vi "helper_fp_print.vi"(1 "VI Path":string, 2 "HTML File Path":string, 3 "Image Directory":string) -> (0 "status":bool, 4 "code":i32, 5 "source":string)   [LabVIEW 2026]
doc: "Print one VI's FRONT PANEL to an HTML file with PNG images. Driven by RunVIAsTopLevel, which can only set STRING controls - paths are built on the diagram."
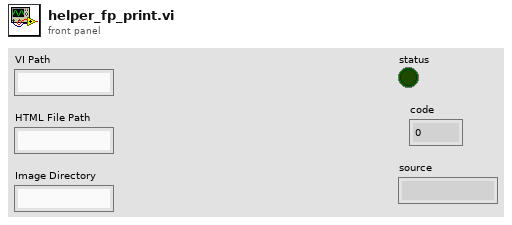
[diagram p1: front panel]
types:
  T1 = enum16{"Custom", "Standard", "Using Panel", "Using SubVI", "Complete"}
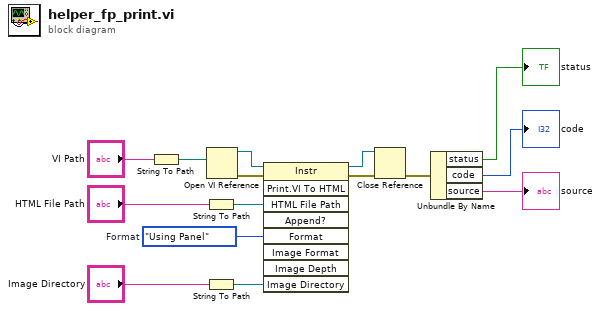
[diagram p0: block diagram]
diagram:
  w8 = T1."Using Panel"  # Format
  n1 = String To Path(string="VI Path") -> (path=w12:path)
  n2 = String To Path(string="HTML File Path") -> (path=w9:path)
  n3 = String To Path(string="Image Directory") -> (path=w7:path)
  n4 = Open VI Reference(vi path=w12) -> (vi reference=w11:refnum<vi>, error out=w10:errorcluster)  [unwired: 5 in]
  n5 = invoke class="Instr" method="Print.VI To HTML"(reference=w11, error in=w10, "HTML File Path"=w9, "Format"=w8, "Image Directory"=w7) -> (reference out=w6:refnum<vi>, error out=w5:errorcluster)  [unwired: 4 in, 7 out]
  n6 = Close Reference(reference=w6, error in (no error)=w5) -> (error out=w4:errorcluster)
  n7 = Unbundle By Name(w4) -> ("status"=→"status":bool, "code"=→"code":i32, "source"=→"source":string)
